vi "SID_test_dump_player.vi"() -> ()   [LabVIEW 2018]
doc: "This VI illustrates how to generate and play sine, square, sawtooth and triangle waveforms. You can change the frequency and type of the waveform generated as it plays continuously."
uses:
  SID_voice_reg.ctl
  SID_filter_reg.ctl
  <vilib>/sound2/lvsound2.llb/Sampling Mode.ctl
  <vilib>/sound2/lvsound2.llb/Sound Data Format.ctl
  <vilib>/sound2/lvsound2.llb/Sound Output Set Volume (Single).vi
  <vilib>/sound2/lvsound2.llb/Sound Output Write (DBL Single).vi
panel:
  in  "Filter":T1 {"vol" format="%0.2f"; "res" format="%0.2f"; "freq" format="%0.2f"}
  in  "VC3":T2 {"Duty" format="%0.2f"; "ADSR"."R" format="%0.2f"; "ADSR"."S" format="%0.2f"; "ADSR"."D" format="%0.2f"; "ADSR"."A" format="%0.2f"; "freq" format="%0.2f"}
  in  "VC1":T2 {"Duty" format="%0.2f"; "ADSR"."R" format="%0.2f"; "ADSR"."S" format="%0.2f"; "ADSR"."D" format="%0.2f"; "ADSR"."A" format="%0.2f"; "freq" format="%0.2f"}
  in  "VC2":T2 {"Duty" format="%0.2f"; "ADSR"."R" format="%0.2f"; "ADSR"."S" format="%0.2f"; "ADSR"."D" format="%0.2f"; "ADSR"."A" format="%0.2f"; "freq" format="%0.2f"}
  out "VC3":dbl[](graph)
  out "VC2":dbl[](graph)
  out "VC1":dbl[](graph)
  out "data size(s)":i32
  out "time Audio":u32
  out "time SID":u32
  in  "Volume":dbl=0.5
  out "Wave":dbl[](graph)
  in  "Stop":bool
  in  "Device ID":u32
  # "D:\\work\\experimets\\C64\\a_mind_is_born_LV.wav"
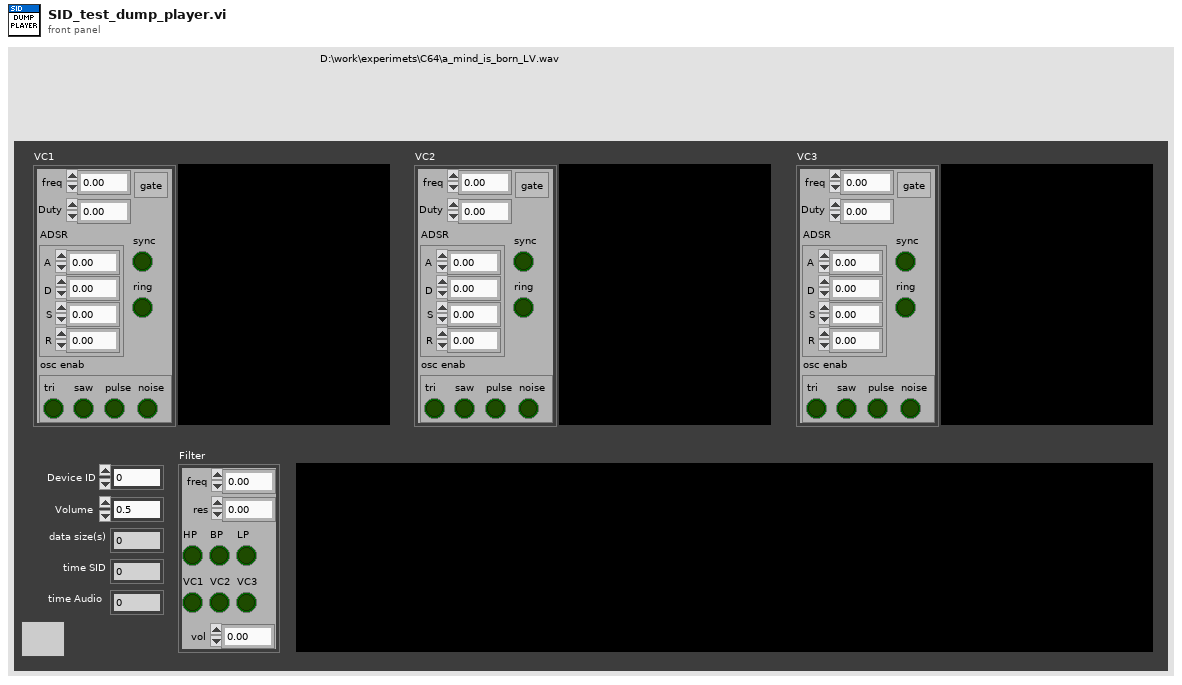
[diagram p1: front panel]
types:
  T1 = typedef "SID_filter_reg.ctl" = cluster{"freq":dbl, "res":dbl, "HP":bool, "BP":bool, "LP":bool, "VC1":bool, "VC2":bool, "VC3":bool, "vol":dbl}
  T2 = typedef "SID_voice_reg.ctl" = cluster{"freq":dbl, "gate":bool, "ADSR":cluster{"A":dbl, "D":dbl, "S":dbl, "R":dbl}, "Duty":dbl, "osc enab":cluster{"tri":bool, "saw":bool, "pulse":bool, "noise":bool}, "sync":bool, "ring":bool}
  T3 = enum16{"idle", "pre-attack", "attack", "pre-decay", "decay", "sustain", "pre-release", "release"}
  T4 = typedef "Sound Data Format.ctl" = cluster{"sample rate (S/s)":dbl, "number of channels":i32, "bits per sample":i32}
  T5 = typedef "Sampling Mode.ctl" = i32
  T6 = typedef "Sound Output Task ID.ctl" = u32
  T7 = cluster{"mod":dbl, "acc":dbl, "counter acc":dbl, "counter":i32}
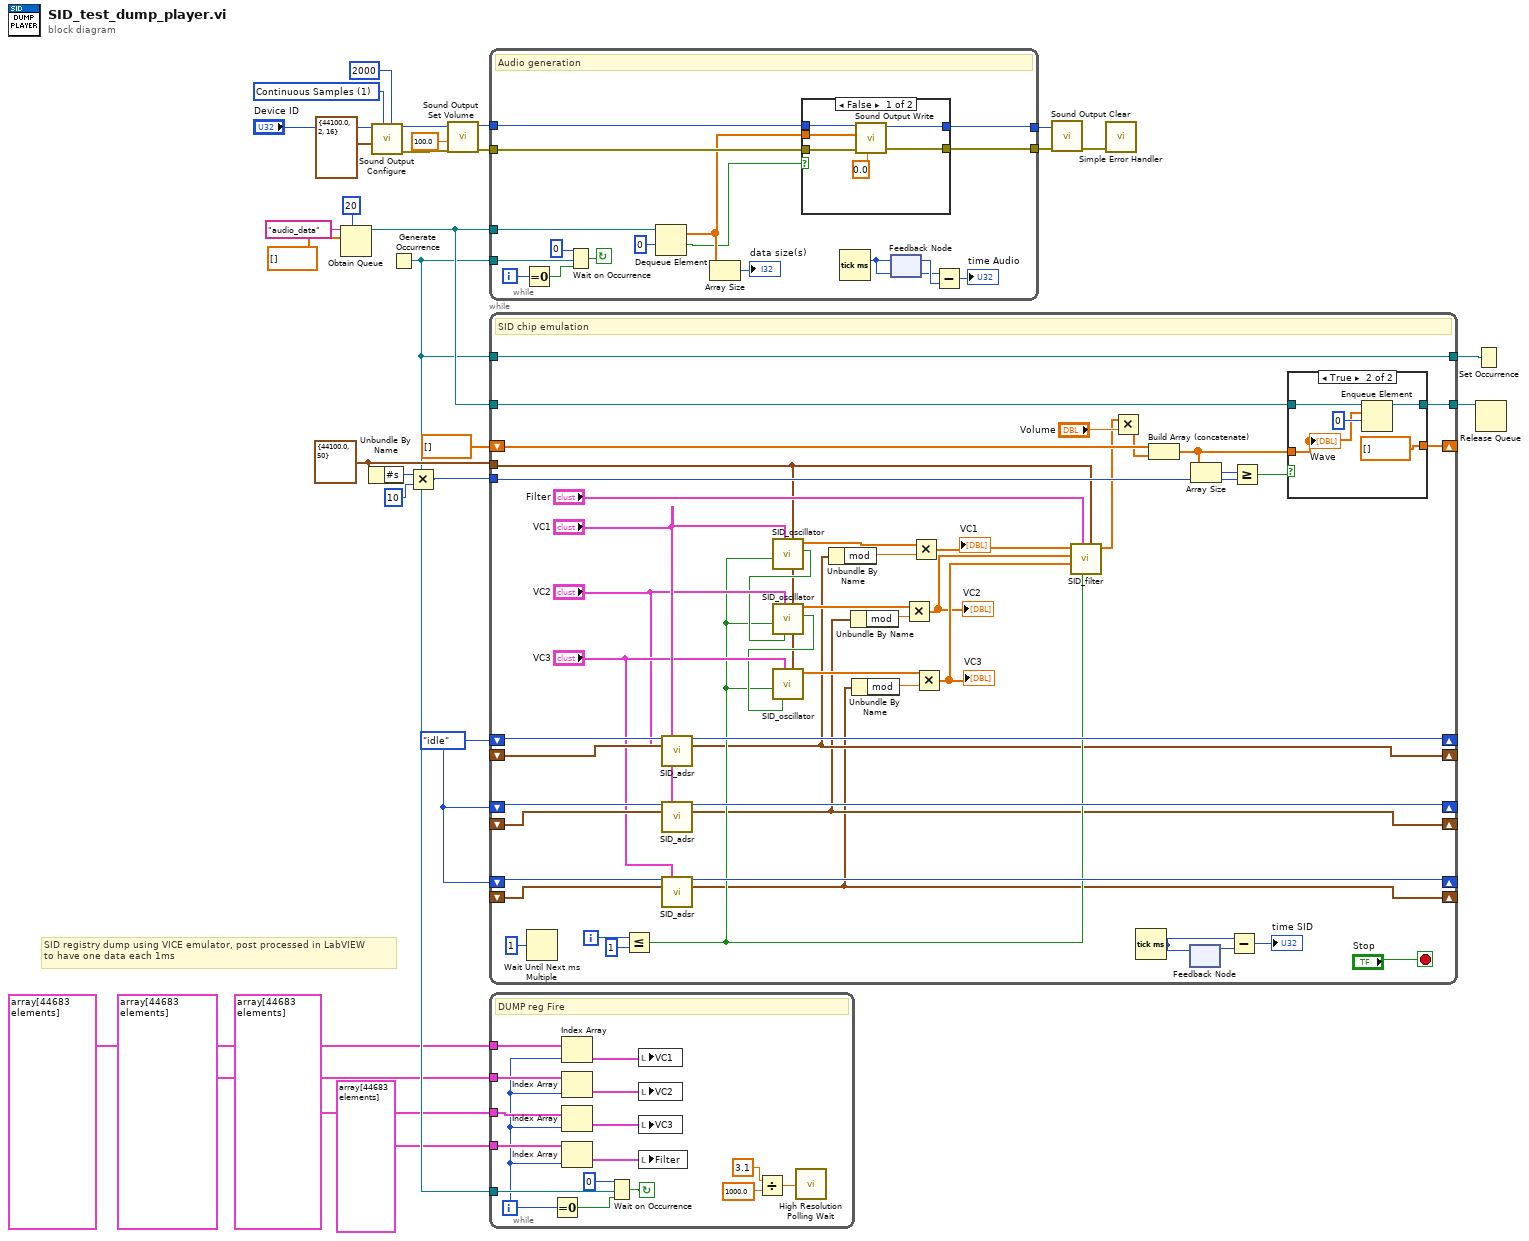
[diagram p0: block diagram]
diagram:
  w9 = cluster{"Fs":dbl, "#s":i32} {"Fs"=44100.0, "#s"=50} ("sampling info")
  w5 = T3."idle"
  w28 = T5 1 items=["Finite Samples", "Continuous Samples"] ("sample mode")
  # "SID registry dump using VICE emulator, post processed in LabVIEW\nto have one data each 1ms"
  n1 = Obtain Queue(max queue size (-1, unlimited)=20, name (unnamed)="audio_data", element data type=dbl[] []) -> (queue out=w16:refnum<queue>)  [unwired: 2 in, 2 out]
  n2 = Unbundle By Name(w9) -> ("#s"=w11:i32)
  n3 = call <vilib>:"Sound Output Configure.vi"("number of samples/ch"=2000 ("Number of Samples/ch"), "sample mode"=w28, "sound format"=T4 {"sample rate (S/s)"=44100.0, "number of channels"=2, "bits per sample"=16} ("Sound Format"), "device ID"="Device ID") -> ("error out"=w25:errorcluster, "task ID"=w23:T6)  [unwired: 6 in]
  n4 = Generate Occurrence() -> (w7:refnum<k4>)
  n5 = Multiply(x=w11, y=10) -> (x*y=w8:i32)
  n6 = call-poly <vilib>:"Sound Output Set Volume.vi"("error in (no error)"=w25, "volume"=100.0, "task ID"=w23) -> ("error out"=w21:errorcluster, "task ID out"=w22:T6)  [unwired: 7 in]
  n7 = while {
    tunnel: w22 -> [w38]
    tunnel: w21 -> [w39]
    tunnel: [w35] -> w20
    tunnel: [w34] -> w19
    tunnel: w7 -> [w46]
    tunnel: w16 -> [w36]
    i -> [w40]
    stop <- w44 continue-if-true
    # "Audio generation"
    n8 = Equal To 0?(x=w40) -> (x = 0?=w32:bool)
    n9 = Wait on Occurrence(1:w32, 2:w46, 3:0 ("ms timeout (-1)")) -> (0:w44:bool)
    n10 = Dequeue Element(queue=w36, timeout in ms (-1)=0) -> (element=w31:dbl[], timed out?=w30:bool)  [unwired: 1 in, 2 out]
    n11 = Array Size(array=w31) -> (size(s)=→"data size(s)":i32)
    n12 = case shown="False" w30 {
      tunnel: w39 -> [w52 w53]
      tunnel: w38 -> [w51 w54]
      tunnel: [w49 w54] -> w35
      tunnel: [w48 w53] -> w34
      tunnel: w31 -> [w47 _]
      frame False {
        n13 = call-poly <vilib>:"Sound Output Write.vi"("timeout (sec)"=0.0, "error in (no error)"=w52, "data"=w47, "task ID"=w51) -> ("error out"=w48:errorcluster, "task ID out"=w49:T6)  [unwired: 6 in]
      }
      frame True {
      }
    }
    n14 = Tick Count (ms)() -> (millisecond timer value=w41:u32)
    n15 = feedback #1() -> (w42:u32)  [unwired: 1 in]
    n16 = feedback-in #1(w41) -> ()
    n17 = Subtract(x=w41, y=w42) -> (x-y=→"time Audio":u32)
  }
  n18 = while {
    shift-right: [w61] -> _
    shift-left: _ -> [w87]
    shift-right: [w86] -> _
    shift-left: w5 -> [w88]
    tunnel: w7 -> [w98]
    tunnel: [w98] -> w18
    tunnel: w16 -> [w95]
    tunnel: [w94] -> w15
    shift-right: [w89] -> _
    shift-left: dbl[] [] -> [w93]
    shift-right: [w58] -> _
    shift-left: _ -> [w83]
    shift-right: [w82] -> _
    shift-left: w5 -> [w84]
    tunnel: w9 -> [w57]
    shift-right: [w56] -> _
    shift-left: _ -> [w80]
    shift-right: [w81] -> _
    shift-left: w5 -> [w79]
    tunnel: w8 -> [w78]
    i -> [w72]
    stop <- "Stop" stop-if-true
    # "SID chip emulation"
    n19 = Wait Until Next ms Multiple(millisecond multiple=u32 1) -> ()  [unwired: 1 out]
    n20 = Less Or Equal?(x=w72, y=1) -> (x <= y?=w62:bool)
    n21 = call "SID_adsr.vi"("status in"=w88, "Reg"="VC1", "acc in"=w87) -> ("status out"=w86:T3, "acc out"=w61:T7)  [unwired: 11 in]
    n22 = call "SID_adsr.vi"("status in"=w84, "Reg"="VC2", "acc in"=w83) -> ("status out"=w82:T3, "acc out"=w58:T7)  [unwired: 11 in]
    n23 = call "SID_adsr.vi"("status in"=w79, "Reg"="VC3", "acc in"=w80) -> ("status out"=w81:T3, "acc out"=w56:T7)  [unwired: 11 in]
    n24 = call "SID_oscillator.vi"("sampling info"=w57, "Reg"="VC1", "reset phase"=w62) -> ("MSB out"=w66:bool, "wave"=w65:dbl[])  [unwired: 7 in]
    n25 = call "SID_oscillator.vi"("sampling info"=w57, "MSB in"=w66, "Reg"="VC2", "reset phase"=w62) -> ("MSB out"=w63:bool, "wave"=w67:dbl[])  [unwired: 6 in]
    n26 = call "SID_oscillator.vi"("sampling info"=w57, "MSB in"=w63, "Reg"="VC3", "reset phase"=w62) -> ("wave"=w64:dbl[])  [unwired: 6 in, 1 out]
    n27 = Unbundle By Name(w61) -> ("mod"=w60:dbl)
    n28 = Unbundle By Name(w58) -> ("mod"=w59:dbl)
    n29 = Unbundle By Name(w56) -> ("mod"=w55:dbl)
    n30 = Multiply(x=w67, y=w59) -> (x*y=w73:dbl[])
    "VC2" <- w73
    n31 = Multiply(x=w65, y=w60) -> (x*y=w76:dbl[])
    "VC1" <- w76
    n32 = Multiply(x=w64, y=w55) -> (x*y=w75:dbl[])
    "VC3" <- w75
    n33 = call "SID_filter.vi"("sampling info"=w57, "reset"=w62, "filter"="Filter", "VC3"=w75, "VC2"=w73, "VC1"=w76) -> ("out"=w77:dbl[])  [unwired: 5 in]
    n34 = Multiply(x=w77, y="Volume") -> (x*y=w85:dbl[])
    n35 = Tick Count (ms)() -> (millisecond timer value=w102:u32)
    n36 = Build Array (concatenate)(w93, w85) -> (w90:dbl[])
    n37 = feedback-in #2(w102) -> ()
    n38 = feedback #2() -> (w101:u32)  [unwired: 1 in]
    n39 = Array Size(array=w90) -> (size(s)=w92:i32)
    n40 = Subtract(x=w102, y=w101) -> (x-y=→"time SID":u32)
    n41 = Greater Or Equal?(x=w92, y=w78) -> (x >= y?=w91:bool)
    n42 = case shown="True" w91 {
      tunnel: w95 -> [w103 w109]
      tunnel: [w103 w108] -> w94
      tunnel: w90 -> [w104 w105]
      tunnel: [w104 dbl[] []] -> w89
      frame False {
      }
      frame True {
        n43 = Enqueue Element(queue=w109, element=w105, timeout in ms (-1)=0) -> (queue out=w108:refnum<queue>)  [unwired: 1 in, 2 out]
        "Wave" <- w105
      }
    }
  }
  n44 = while {
    tunnel: w7 -> [w123]
    tunnel: T1[] array[44683 elements] ("filter") -> [w121]
    tunnel: T2[] array[44683 elements] ("Array") -> [w120]
    tunnel: T2[] array[44683 elements] ("voice 2") -> [w119]
    tunnel: T2[] array[44683 elements] ("voice 1") -> [w122]
    i -> [w118]
    stop <- w117 continue-if-true
    # "DUMP reg Fire"
    n45 = Equal To 0?(x=w118) -> (x = 0?=w124:bool)
    n46 = Index Array(array=w122, index=w118) -> (element=w116:T2)
    n47 = Index Array(array=w119, index=w118) -> (element=w115:T2)
    n48 = Index Array(array=w120, index=w118) -> (element=w110:T2)
    n49 = Index Array(array=w121, index=w118) -> (element=w114:T1)
    n50 = Wait on Occurrence(1:w124, 2:w123, 3:0 ("ms timeout (-1)")) -> (0:w117:bool)
    n51 = local write "VC1"(w116) -> ()
    n52 = local write "VC2"(w115) -> ()
    n53 = local write "VC3"(w110) -> ()
    n54 = local write "Filter"(w114) -> ()
    n55 = Divide(x=3.1 ("mseconds to wait"), y=1000.0) -> (x/y=w112:dbl)
    n56 = call <vilib>:"High Resolution Polling Wait.vi"("seconds to wait"=w112) -> ()  [unwired: 10 in, 1 out]
  }
  n57 = call <vilib>:"Sound Output Clear.vi"("error in (no error)"=w19, "task ID"=w20) -> ("error out"=w26:errorcluster)  [unwired: 9 in]
  n58 = call <vilib>:"Simple Error Handler.vi"("error in (no error)"=w26) -> ()  [unwired: 4 in, 5 out]
  n59 = Set Occurrence(w18) -> ()
  n60 = Release Queue(queue=w15) -> ()  [unwired: 2 in, 3 out]
